vi "test_OneSessOnePinGroupOneInstrOneSiteReservation_CallNiDcPowerGetConnections1PinMConnections_ReturnsTwoConnections.vi"() -> (6 "pass":bool, 8 "result":string, 15 "error out":errorcluster)   [LabVIEW 2021, in "MeasurementServerTests.lvlib"]
uses:
  MeasurementServerTests.lvlib
  Runtime/Sessions/niDCPower/Connection with Session.ctl
  Runtime/Clients/Session Management V1/Session Reservation/Connection.ctl
  0bcc7825-b361-4d47-8536-1ed12f6e0935.vi
  <vilib>/AdvancedString/1D String Array to Delimited String.vi
  0bcc7825-b361-4d47-8536-1ed12f6e0935.vi/94283ac5-2298-4b3a-b57d-7be67da3787d.vi
  0bcc7825-b361-4d47-8536-1ed12f6e0935.vi/f7d9c9cb-0251-4d67-81cb-70e1b0e8b69f.vi
  0bcc7825-b361-4d47-8536-1ed12f6e0935.vi/48d9c053-c3ce-4ae4-8653-846fcb37df32.vi
  0bcc7825-b361-4d47-8536-1ed12f6e0935.vi/38a8d12d-9165-42a0-bd04-ad62bed472d1.vi
  Runtime/Sessions/niDCPower/Get Connections - 1Pin MConn.vi
  <vilib>/JDP Science/JSONtext/Variant to JSON Text.vi
  <vilib>/JDP Science/JSONtext/LVClass Serializer/JSONtext LVClass Serializer.lvclass
  Runtime/Sessions/niDCPower/NI Session Management niDCPower.lvlib
  Runtime/Clients/Session Management V1/Session Reservation/Session Reservation.lvclass
panel:
  in  "error in":errorcluster
  # "Test assumes discovery service, pin map service, and session management service have already been started."
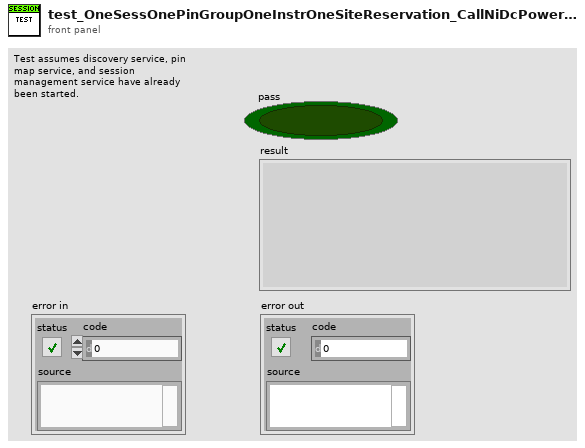
[diagram p1: front panel]
types:
  T1 = typedef "NI Session Management niDCPower.lvlib/Connection with Session.ctl" = cluster{"connection":T2, "session":refnum<k15>}
  T2 = typedef "NI Session Management V1 Client.lvlib/Session Reservation.lvclass/Connection.ctl" = cluster{"pin or relay name":string, "site":i32, "instrument type id":string, "channel":string}
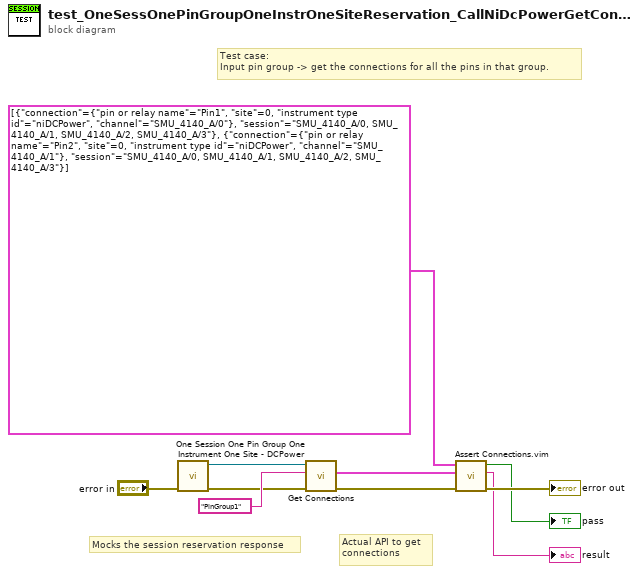
[diagram p0: block diagram]
diagram:
  # "Actual API to get\nconnections"
  # "Mocks the session reservation response"
  # "Test case:\nInput pin group -> get the connections for all the pins in that group."
  n1 = call "One Session One Pin Group One Instrument One Site - DCPower.vi"("error in"="error in") -> ("error out"=w1:errorcluster, "session reservation out"=w3:refnum<class "Session Reservation.lvclass">)  [unwired: 9 in]
  n2 = call-poly "Get Connections.vi"("error in"=w1, "pin or relay name"="PinGroup1", "session reservation in"=w3) -> ("error out"=w9:errorcluster, "connections"=w4:T1[])  [unwired: 6 in, 1 out]
  n3 = call "Assert Connections.vim"("error in"=w9, "actual connections"=w4, "expected connections"=T1[] [{"connection"={"pin or relay name"="Pin1", "site"=0, "instrument type id"="niDCPower", "channel"="SMU_4140_A/0"}, "session"="SMU_4140_A/0, SMU_4140_A/1, SMU_4140_A/2, SMU_4140_A/3"}, {"connection"={"pin or relay name"="Pin2", "site"=0, "instrument type id"="niDCPower", "channel"="SMU_4140_A/1"}, "session"="SMU_4140_A/0, SMU_4140_A/1, SMU_4140_A/2, SMU_4140_A/3"}] ("appended array")) -> ("error out"=→"error out":errorcluster, "result"=→"result":string, "pass"=→"pass":bool)  [unwired: 6 in]
